vi "Calculate_DNL_DAC.vi"(8 "error in":errorcluster, 9 "DUT Range (pk-pk)":dbl=2.0, 10 "Resolution (bits)":i32=12, 11 "DAC Code Voltage":dbl[](array[numeric])) -> (0 "error out":errorcluster, 1 "Min DNL":dbl, 2 "Max DNL":dbl, 3 "DNL Data":dbl[](graph))   [LabVIEW 2026, in "Core.lvlib"]
uses:
  Core.lvlib
panel:
  out "Min Index":i32
  out "Max Index":i32
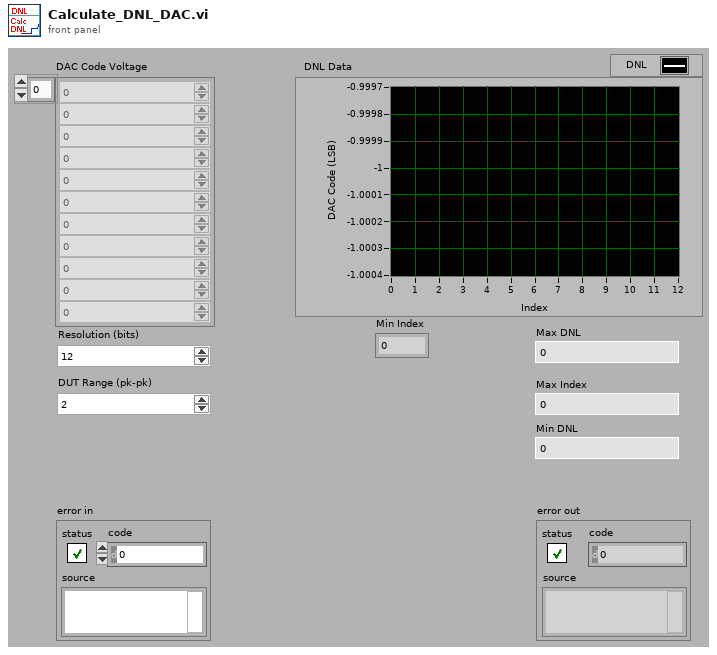
[diagram p1: front panel]
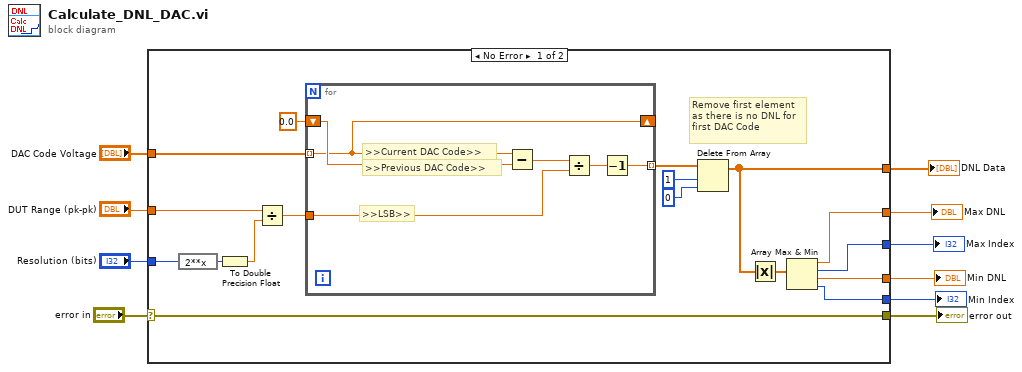
[diagram p0: block diagram]
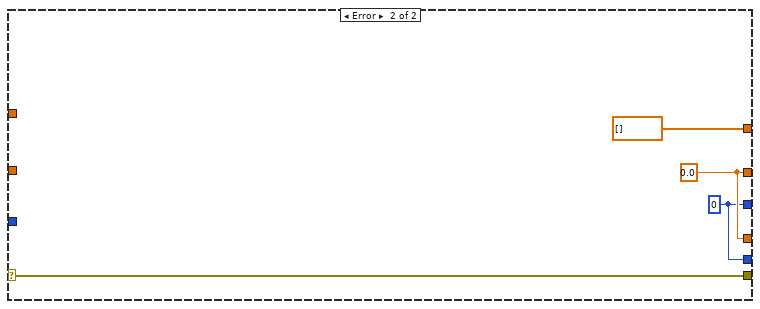
[diagram p2: hidden frame]
diagram:
  n1 = case shown="No Error" "error in" {
    selector: "error in" -> [w11 w34]
    tunnel: "DAC Code Voltage" -> [w27 _]
    tunnel: "DUT Range (pk-pk)" -> [w26 _]
    tunnel: [w20 dbl[] []] -> w8
    tunnel: [w18 w36] -> w7
    tunnel: [w17 w35] -> w6
    tunnel: "Resolution (bits)" -> [w16 _]
    tunnel: [w14 w36] -> w4
    tunnel: [w13 w35] -> w3
    tunnel: [w11 w34] -> w2
    frame No Error {
      # "Remove first element\nas there is no DNL for\nfirst DAC Code"
      n2 = expression code="2**x"(w16) -> (w15:i32)
      n3 = To Double Precision Float(number=w15) -> (double precision float=w12:dbl)
      n4 = Divide(x=w26, y=w12) -> (x/y=w25:dbl)
      n5 = for {
        tunnel: w27 -> [w32] mode=indexing
        tunnel: w25 -> [w30]
        shift-right: [w32] -> _
        shift-left: 0.0 ("Numeric") -> [w33]
        tunnel: [w28] -> w23 mode=indexing
        # ">>LSB>>"
        # ">>Previous DAC Code>>"
        # ">>Current DAC Code>>"
        n6 = Subtract(x=w32, y=w33) -> (x-y=w31:dbl)
        n7 = Divide(x=w31, y=w30) -> (x/y=w29:dbl)
        n8 = Decrement(x=w29) -> (x-1=w28:dbl)
      }
      n9 = Delete From Array(array=w23, length=1, index=0) -> (array with subset deleted=w20:dbl[])  [unwired: 1 out]
      n10 = Absolute Value(x=w20) -> (abs(x)=w19:dbl[])
      n11 = Array Max & Min(array=w19) -> (max value=w18:dbl, max index (indices)=w17:i32, min value=w14:dbl, min index (indices)=w13:i32)
    }
    frame Error {
      w35 = 0
      w36 = 0.0
    }
  }
  "error out" <- w2
  "DNL Data" <- w8
  "Max DNL" <- w7
  "Max Index" <- w6
  "Min DNL" <- w4
  "Min Index" <- w3
